vi "Motor and Elevator Testbench.vi"() -> ()   [LabVIEW 2021]
uses:
  Elevator/Elevator.lvclass
  Motor/Motor.lvclass
panel:
  in  "Elevator Control":dbl
  in  "Motor Control":dbl
  in  "stop":bool
  out "Actual Position":dbl
  out "error out":errorcluster
  out "Actual Torque":dbl
  out "Actual Speed":dbl
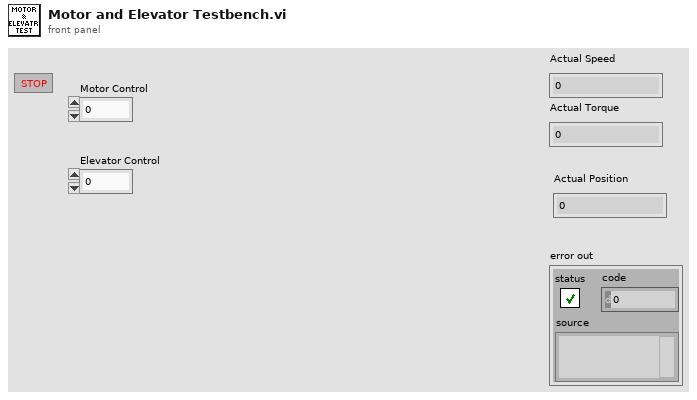
[diagram p1: front panel]
types:
  T1 = typedef "Device Context Cluster.ctl" = cluster{"Motor in":refnum<class "Motor.lvclass">, "Elevator.lvclass":refnum<class "Elevator.lvclass">}
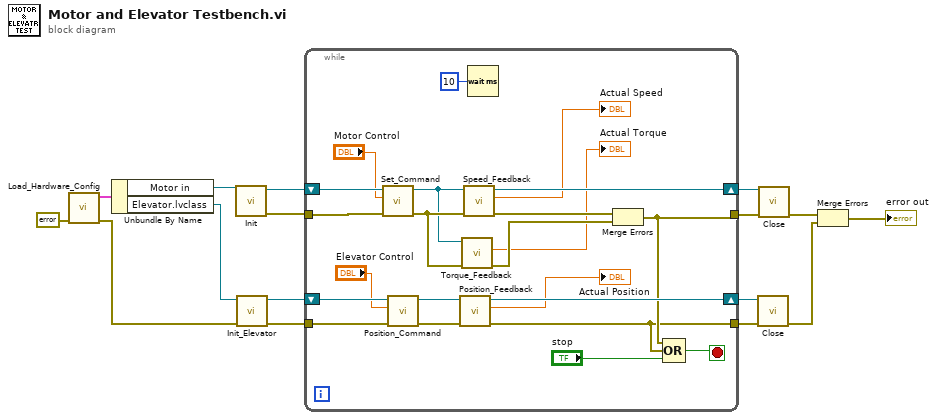
[diagram p0: block diagram]
diagram:
  n1 = call "Load_Hardware_Config.vi"("error in (no error)"=errorcluster {"status"=FALSE, "code"=0, "source"=""}) -> ("error out"=w13:errorcluster, "Device Context Cluster"=w16:T1)  [unwired: 9 in]
  n2 = Unbundle By Name(w16) -> ("Motor in"=w14:refnum<class "Motor.lvclass">, "Elevator.lvclass"=w15:refnum<class "Elevator.lvclass">)
  n3 = call "Init.vi"("Motor in"=w14) -> ("error out"=w10:errorcluster, "Motor out"=w11:refnum<class "Motor.lvclass">)  [unwired: 9 in]
  n4 = call "Init_Elevator.vi"("error in (no error)"=w13, "Elevator in"=w15) -> ("error out"=w3:errorcluster, "Elevator out"=w4:refnum<class "Elevator.lvclass">)  [unwired: 8 in]
  n5 = while {
    shift-right: [w38] -> w9
    shift-left: w11 -> [w24]
    shift-right: [w33] -> w1
    shift-left: w4 -> [w20]
    tunnel: w10 -> [w26]
    tunnel: [w31] -> w8
    tunnel: w3 -> [w21]
    tunnel: [w30] -> w2
    stop <- w28 stop-if-true
    n6 = call "Set_Command.vi"("error in (no error)"=w26, "Motor Control"="Motor Control", "Motor in"=w24) -> ("error out"=w25:errorcluster, "Motor out"=w23:refnum<class "Motor.lvclass">)  [unwired: 7 in]
    n7 = call "Position_Command.vi"("error in (no error)"=w21, "Elevator Position Control"="Elevator Control", "Elevator in"=w20) -> ("error out"=w18:errorcluster, "Elevator out"=w19:refnum<class "Elevator.lvclass">)  [unwired: 7 in]
    n8 = call-dynamic "Position_Feedback.vi"("error in (no error)"=w18, "Elevator in"=w19) -> ("error out"=w30:errorcluster, "Actual Position"=→"Actual Position":dbl, "Elevator out"=w33:refnum<class "Elevator.lvclass">)  [unwired: 7 in]
    n9 = call "Torque_Feedback.vi"("error in (no error)"=w25, "Motor in"=w23) -> ("error out"=w35:errorcluster, "Actual Torque"=→"Actual Torque":dbl)  [unwired: 7 in, 1 out]
    n10 = call "Speed_Feedback.vi"("error in (no error)"=w25, "Motor in"=w23) -> ("error out"=w36:errorcluster, "Actual Speed"=→"Actual Speed":dbl, "Motor out"=w38:refnum<class "Motor.lvclass">)  [unwired: 7 in]
    n11 = Wait (ms)(milliseconds to wait=u32 10) -> ()  [unwired: 1 out]
    n12 = Merge Errors(w36, w35) -> (w31:errorcluster)
    n13 = Compound Arithmetic op=OR(w31, w30, "stop") -> (w28:bool)
  }
  n14 = call-dynamic "Close.vi"("error in (no error)"=w2, "Elevator in"=w1) -> ("error out"=w5:errorcluster)  [unwired: 8 in, 1 out]
  n15 = call "Close.vi"("error in (no error)"=w8, "Motor in"=w9) -> ("error out"=w7:errorcluster)  [unwired: 8 in, 1 out]
  n16 = Merge Errors(w7, w5) -> (→"error out":errorcluster)
